vi "AlliGator Phasor Graph Panel.vi"() -> ()   [LabVIEW 2021, in "AlliGator Phasor Graph.lvlib"]
uses:
  AlliGator Phasor Graph.lvlib
  Phasor/Phasor Calibration Type.ctl
  Phasor/Phasor (g, s).ctl
  Phasor/Phasor (m, phi).ctl
  AlliGator Phasor Graph Ctrl Refnums.ctl
  Globals, Variables, Constants/AlliGator Refnums List.ctl
  Settings/AlliGator Settings List.ctl
  Action Engine/AlliGator Q Element.ctl
  Action Engine/AlliGator Q Event.ctl
  Graphs/XY Graph/XY Graph Event.ctl
  <vilib>/Utility/miscctls.llb/LVPoint32TypeDef.ctl
  Globals, Variables, Constants/AlliGator Variables List.ctl
  Variant/Variant to Data/Variant to Boolean.vi
  Settings/AlliGator Settings+.lvlib
  Variant/Variant to Data/Variant to Data.lvlib
  Notebook/Notebook.lvlib
  Action Engine/AlliGator Action Engine.lvlib
  GUI/GUI.lvlib
  GUI/AlliGator GUI.lvlib
  Error/Error.lvlib
  Graphs/XY Graph/XY Graph Add-Ons.lvlib
  Python Plugins API/AlliGator Python Plugins.lvlib
  Decay Analysis/Decay Processing/AlliGator Decay Processing.lvlib
  Phasor Calibration/AlliGator Phasor Calibration.lvlib
  Phasor/Phasor.lvlib
  Globals, Variables, Constants/AlliGator Globals, Variables & Constants.lvlib
  Utilities/Utilities.lvlib
panel:
  in  "Refresh SEPL":bool
  in  "Calibration Type":T1
  in  "Phasor Graph Active":bool
  in  "Phasor Graph Frequency":dbl[unit]=80000000.0 caption="Phasor Frequency"
  in  "Calibration Lifetime":dbl[unit] min=0.0
  in  "Pin Button":bool=TRUE
  out "Phasor Graph TipStrip":string caption="Lifetime Graph TipStrip"
  out "Phasor Graph":cluster{"X Array":dbl[], "Y Array":dbl[]}[](graph)
  in  "Phasor Reference 2 Control":dbl(c297)
  out "Phase Lifetime 2":dbl[unit]=nan format="%#.3g"
  out "Average Lifetime SDV":dbl[unit]=nan caption="+/-" format="%#.3g"
  out "Phasor Ratio SDV":dbl=nan caption="+/-" format="%#.3g"
  out "Modulus Lifetime SDV":dbl[unit]=nan caption="+/-" format="%#.3g"
  out "Phase Lifetime SDV":dbl[unit]=nan caption="+/-" format="%#.3g"
  out "Phasor Graph Average Lifetime":dbl[unit]=nan caption="<tau>_a" format="%#.3g"
  out "Phasor Graph Phasor Ratio":dbl=nan caption="Amplitude Ratio (a1)" format="%#.3g"
  out "Phasor Graph Modulus Lifetime":dbl[unit]=nan caption="Modulus Lifetime" format="%#.3g"
  in  "Current Phasor (m, phi)":T2={"m"=nan, "phi"=nan} {"phi" format="%#_4g"; "m" format="%#_4g"}
  in  "Phasor Reference 1 Control":dbl(c297)
  out "Phase Lifetime 1":dbl[unit]=nan format="%#.3g"
  out "Phasor Graph Phase Lifetime":dbl[unit]=nan caption="Phase Lifetime" format="%#.3g"
  in  "Current Phasor (g, s)":T3={"g"=nan, "s"=nan} caption="Current Phasor" {"s" format="%#_4g"; "g" format="%#_4g"}
  in  "Save Phasor Graph Image":bool
  in  "Single Step Phasor":bool
  in  "Phasor Frame Slide":i32(slide) caption="Phasor Frame Slider" min=0 step=1 scale=1.0..1.1
  in  "Show Line":bool
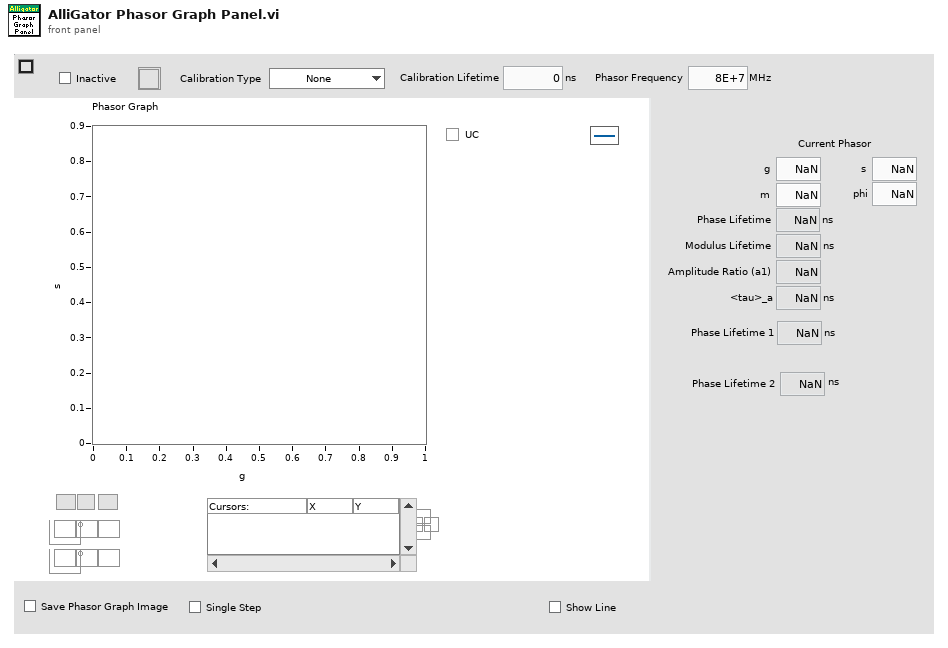
[diagram p1: front panel]
types:
  T1 = typedef "Phasor.lvlib/Phasor Calibration Type.ctl" = enum16{"None", "Single Phasor", "Phasor Series", "Phasor Map"}
  T2 = typedef "Phasor.lvlib/Phasor (m, phi).ctl" = cluster{"m":dbl, "phi":dbl}
  T3 = typedef "Phasor.lvlib/Phasor (g, s).ctl" = cluster{"g":dbl, "s":dbl}
  T4 = typedef "AlliGator GUI.lvlib/AlliGator Refnums List.ctl" = enum16{"---------- AlliGator Control Refnums ----------", "AlliGator Tab Control Refnum", "Dataset Ctrl Refnums", "Image Histogram Ctrl Refnums", "Intensity Time Trace Ctrl Refnums", "Decay Graph Ctrl Refnums", "Decay Statistics Graph Ctrl Refnums", "Phasor Graph Ctrl Refnums", "Phasor Ratio Graph Ctrl Refnums", "Phasor Plot Ctrl Refnums", "Lifetime & Other Parameters Ctrl Refnums", "Decay Fit Parameter Map Ctrl Refnums", "Parameter Map Ctrl Refnums", "Other AlliGator Ctrl Refnums", "---------- AlliGator Menu Refnums ----------", "AlliGator Menu", "---------- IO Device ID ----------", "Mouse ID", "Keyboard ID"}
  T5 = typedef "AlliGator Phasor Graph.lvlib/AlliGator Phasor Graph Ctrl Refnums.ctl" = cluster{"Phasor Ratio":refnum<vi>, "Modulus Lifetime":refnum<vi>, "Phasor at cursor (m, phi)":refnum<vi>, "Phase Lifetime":refnum<vi>, "Phasor at cursor (g, s)":refnum<vi>, "Phasor Graph Average Lifetime":refnum<vi>, "Phasor Graph Active":refnum<vi>, "Save Phasor Graph":refnum<vi>, "Phasor Frame Slide":refnum<vi>, "Single Step Phasor":refnum<vi>, "Calibration Type":refnum<vi>, "Show Line":refnum<vi>, "Phase Lifetime 1":refnum<vi>, "Phase Lifetime 2":refnum<vi>, "Phasor Graph Frequency":refnum<vi>, "Phasor Reference 1 Control":refnum<vi>, "Phasor Reference 2 Control":refnum<vi>, "Calibration Lifetime":refnum<vi>, "Phase Lifetime SDV":refnum<vi>, "Average Lifetime SDV":refnum<vi>, "Phasor Ratio SDV":refnum<vi>, "Modulus Lifetime SDV":refnum<vi>, "Phasor Graph":refnum<vi>}
  T6 = cluster{"Event Registration Refnum":refnum<event-registration>, "Event Registration Refnum":refnum<event-registration>}
  T7 = typedef "AlliGator Settings+.lvlib/AlliGator Settings List.ctl" = enum16{"GUI:Visible Settings Tab", "GUI:Last Run Version", "Source Image:Use Image Histogram for Contrast", "Source Image:Low Count Pixels Rejection Options", "Source Image:High Count Pixels Rejection Options", "Source Image:Use Image Brightness", "Source Image:Blend Overlay with Image Background", "Source Image:Use Fixed ROI Diameter", "Source Image:ROI Diameter", "Source Image:ROI Center Color", "Source Image:Peak Threshold", "Source Image:Intensity Threshold", "Source Image:Image Binning Options", "Source Image:Image Smoothing Options", "Source Image:Image Histogram Active", "Source Image:Invert Binary Mask", "Source Image:Hot Pixel Removal", "Source Image:Overlay Analyzed ROI Center", "Source Image:Auto-Adjust Contrast", "Source Image:Histogram Lower Percentile", "Source Image:Histogram Upper Percentile", "Source Image:Lock ROI with Maps", "Source Image:Save Source Image", "Source Image:Scale Bar Options", "Source Image:Image Resolution (Pixel Size)", "Source Image:Flatfield Correction", "Source Image:Show Dead Left Columns Correction", "Source Image:Dead Left Columns Correction", "Source Image:Image Pre-Processing Operations Order", "Source Image:Overlay ROI Median", "Source Image:Median Overlay Color", "Data Information:Gate Width", "Data Information:Nanotime Gate Separation", "Data Information:Macrotime Gate Separation", "Data Information:Gate Step", "Data Information:# Gates", "Data Information:Gate Image Exposure", "Data Information:Gate Image Integration", "Data Information:Gates to Skip", "Data Information:Gates to Keep", "Data Information:Define Gates to", "Data Information:Channel Name", "Data Information:Available Channel Names", "Data Information:Channel Arithmetic", "Data Information:Background File Subtraction", "Data Information:Background File", "Data Information:Background Scaling Factor", "Data Information:Background Pile-up Correction", "Data Information:Background Pixel Well Capacity", "Data Information:Laser Period", "Data Information:SYNC Period", "Data Information:Pile-up Correction", "Data Information:Pixel Well Capacity", "Data Information:Dataset Scaling Factor", "Fluorescence Decay_Decay Pre-Processing:Reverse Gates", "Fluorescence Decay_Decay Pre-Processing:Verbose Decay Pre-Processing", "Fluorescence Decay_Decay Pre-Processing:Use Decay Pre-Processing", "Fluorescence Decay_Decay Pre-Processing:Background Subtraction", "Fluorescence Decay_Decay Pre-Processing:Background Definition Range", "Fluorescence Decay_Decay Pre-Processing:Baseline Subtraction Method", "Fluorescence Decay_Decay Pre-Processing:Decay Pre-Processing Operations Order", "Fluorescence Decay_Decay Pre-Processing:Smoothing Parameter", "Fluorescence Decay_Decay Pre-Processing:Shift Decay", "Fluorescence Decay_Decay Pre-Processing:Decay Shift Parameters", "Fluorescence Decay_Decay Pre-Processing:Fold Decay", "Fluorescence Decay_Decay Pre-Processing:# Folds", "Fluorescence Decay_Decay Pre-Processing:1-Normalize Decay", "Fluorescence Decay_Decay Pre-Processing:[0-1]-Normalize Decay", "Fluorescence Decay_Decay Pre-Processing:Smoothen Decay", "Fluorescence Decay_Decay Pre-Processing:Extrapolate Decay", "Fluorescence Decay_Decay Pre-Processing:Use Periodicity", "Fluorescence Decay_Decay Pre-Processing:Use Cursors", "Fluorescence Decay_Decay Pre-Processing:Tail Fraction", "Fluorescence Decay_Decay Pre-Processing:Head Fraction", "Fluorescence Decay_Decay Pre-Processing:Additional Points", "Fluorescence Decay_Decay Pre-Processing:Straighten Decay", "Fluorescence Decay_Decay Pre-Processing:Constant Background", "Fluorescence Decay_Decay Pre-Processing:Pixel-Normalize Decay", "Fluorescence Decay_Advanced Analysis:Extract IRF instead of Decay", "Fluorescence Decay_Advanced Analysis:IRF Extraction Options", "Fluorescence Decay_Advanced Analysis:IRF Optimization Options", "Fluorescence Decay_Advanced Analysis:Square Pulse Options", "Fluorescence Decay_Advanced Analysis:IRF Order", "Fluorescence Decay_Advanced Analysis:IRF Time Constants", "Fluorescence Decay_Advanced Analysis:Wavelet Analysis Options", "Fluorescence Decay_Advanced Analysis:Average Lifetime Options", "Fluorescence Decay_Fit Options:Fit Options", "Fluorescence Decay_Fit Options:Use Legacy Fitting Approach", "Fluorescence Decay_Fit Options:Use Data Information Laser Period", "Fluorescence Decay_Fit Parameters:Displayed Fit Parameters", "Fluorescence Decay_Fit Parameters:Fit Parameter Constraints", "Fluorescence Decay_Fit Parameters:Export Tabulated Results", "Fluorescence Decay_Fit Parameters:MLE Baseline Offset Type", "Fluorescence Decay_Fit Parameters:MLE Baseline Offset", "Fluorescence Decay_Fit Parameters:Guess Parameter Names", "Fluorescence Decay_Fit Parameters:Guess Parameter Values", "Fluorescence Decay_Fit Parameters:Guess Parameters Options", "Fluorescence Decay_Fit Parameters:Optimal Offset Selection Criterion", "Fluorescence Decay_Styles:Show Last Decay Only", "Fluorescence Decay_Styles:Decay Graph Color Array", "Fluorescence Decay:Decay Graph Active", "Fluorescence Decay Statistics:Min Peak Value", "Fluorescence Decay Statistics:Reject Low Decay Peak Pixels", "Fluorescence Decay Statistics:Reject High Decay Peak Pixels", "Fluorescence Decay Statistics:Max Peak Value", "Time Traces:Use File Timestamp", "Time Traces:Time Step", "Time Traces:Use Intensity Correction File", "Time Traces:Intensity Correction File", "Phasor Plot:Phasor Plot Smoothing Options", "Phasor Plot:Phasor Plot Size", "Phasor Plot:Phasor Plot Graphics Options", "Phasor Plot:Cumulative Phasor Plot", "Phasor Plot:Use Phasor Brightness", "Phasor Plot:Blend Overlay with Phasor Background", "Phasor Plot:Save Phasor Plot", "Phasor Plot:Show References", "Phasor Plot:Phasor Ratio Decay Range", "Phasor Plot:Exponential Fading", "Phasor Plot:Phasor Ratio Reference Colors", "Phasor Plot:Reference Radius", "Phasor Plot:Show Color Map Vertices", "Phasor Plot:Phasor Plot Active", "Phasor Plot:Phasor Ratio Color Map Type", "Phasor Plot:Phasor Ratio Color Map", "Phasor Plot:Phasor Ratio Display Range", "Phasor Plot:Selected Image ROI(s)", "Phasor Plot:All Image ROIs", "Phasor Plot:Selected Phasor Plot ROI(s)", "Phasor Plot:All Phasor Plot ROIs", "Phasor Plot:Phasor Ratio Color-Coded Quantity", "Phasor Plot:Store Phasor Harmonics", "Phasor Plot:Draw Reference Segment", "Phasor Plot:User-Defined Quantity", "Phasor Plot:Color Scale High Color", "Phasor Plot:Color Scale Low Color", "Phasor Plot:Intensity-weighted Phasor Plot", "Phasor Graph:Phasor Frequency", "Phasor Graph:Phasor Ratio Type", "Phasor Graph:Pixel-level Phasor Computation", "Phasor Graph:Save Phasor Graph", "Phasor Graph:Phasor Graph Active", "Phasor Graph:Phasor SDV Options", "Phasor Graph:Intensity-weighted Phasor Graph", "Phasor Graph:Define Shortest Lifetime as", "Phasor Calibration:Use Backup Calibration if needed", "Phasor Calibration:Backup Calibration Type", "Phasor Calibration:Calibration Type", "Phasor Calibration:Calibration Lifetime", "Phasor Calibration:Calibration Map Algorithm", "Single-Exponential Phasor Locus (SEPL):Gate Parameters", "Single-Exponential Phasor Locus (SEPL):User-defined Gate", "Single-Exponential Phasor Locus (SEPL):User-defined IRF", "Single-Exponential Phasor Locus (SEPL):Phasor Parameters", "Single-Exponential Phasor Locus (SEPL):Decay & IRF Parameters", "Single-Exponential Phasor Locus (SEPL):Display Parameters", "Lifetime Analysis:Decay Analysis Parameters", "Lifetime Analysis:Lifetime Map Active", "Plugins:Python Settings", "Miscellaneous:Verbose Mode", "Miscellaneous:Beep after Script", "Miscellaneous:Saved Image File Format", "Miscellaneous:Exported Gate Image Settings", "Miscellaneous:Include Loading in Timing", "Miscellaneous:Verbose Settings Mode", "Miscellaneous:Histogram Options", "Miscellaneous:Beep on Error", "Miscellaneous:# Logical Processors Used", "Miscellaneous:ROI Description Max Characters", "Miscellaneous:Verbose Error Mode", "Miscellaneous:Transparent Mask Color"}
  T8 = typedef "AlliGator Action Engine.lvlib/AlliGator Q Element.ctl" = cluster{"AlliGator Q Event":T9, "Data":variant}
  T9 = typedef "AlliGator Action Engine.lvlib/AlliGator Q Event.ctl" = enum16{"---- Files ----", "Files:Set Batch Export Files To Save", "Files:Set Dataset Loading & Pre-processing Options", "Files:Check #Frames in Dataset", "Files:Increment Frame Index", "Files:Open Mask Image", "Files:Open White Light Image", "Files:Open Single Dataset", "Files:New Folder of Folders Selected", "Files:Load File (all Types)_Scriptable", "Files:Move Flattened Series to Folders Series", "Files:Select Folder", "Files:Load FLI Dataset", "Files:Load Swiss SPAD 1 Dataset", "Files:Load Swiss SPAD 2 Dataset", "Files:Load .sdt FLI Dataset", "Files:Load .ptu FLI Dataset", "Files:Load .bin FLI Dataset", "Files:Load Single Gate Image Folder", "Files:Load I/m/phi Dataset (deprecated)", "Files:Load Single Image", "Files:Subtract Background File", "Files:Export FLI Dataset", "Files:Load HDF5 FLI Dataset", "Files:Set Destination File Path", "Files:Save Mask Image", "Files:Batch Conversion", "Files:New Folder Selected", "Files:Close FLI Dataset", "Files:Close FLI Dataset Series", "Files:Close White Light Image", "Files:Close Mask Image", "---- FLI Dataset ----", "FLI Dataset:Channel Arithmetic", "FLI Dataset:Export Average Lifetime Map as ASCII", "FLI Dataset:Export User-Defined Quantity Map as ASCII", "FLI Dataset:Python Function FLI Dataset Event", "FLI Dataset:ROI Analysis", "FLI Dataset:Tilted Logistic Square Gated IRF Characteristics Map", "FLI Dataset:Logistic Square Gated IRF Characteristics Map", "FLI Dataset:Square Gated IRF Characteristics Map", "FLI Dataset:Multi-ROI Single-Pixel Phasor Analysis", "FLI Dataset:Multi-ROI Single-Pixel NLSF Analysis", "FLI Dataset:All ROIs IRF Extraction", "FLI Dataset:All ROIs Decay Fit Non-Interactive (Fast + Individual IRF)", "FLI Dataset:All ROIs Phasor Analysis", "FLI Dataset:All ROIs Decay Fit", "FLI Dataset:Fluorescence Decay Statistics", "FLI Dataset:Update Decay Statistics Graph", "FLI Dataset:Get Decay from ROI", "FLI Dataset:All ROIs Average Lifetimes", "FLI Dataset:Save/Load Local IRFs", "FLI Dataset:Clear Local IRFs", "FLI Dataset:Phasor Calibration Maps (# Gates Series) Script", "FLI Dataset:Calibrated Phasor Map Series", "---- FLI Dataset Series ----", "FLI Dataset Series:Sum All Datasets in Series", "FLI Dataset Series:Add Dataset to Accumulated Dataset", "FLI Dataset Series:Display Accumulated Dataset", "FLI Dataset Series:Clear Dataset Series Sum", "FLI Dataset Series:Time-Series Analysis (NLSF)", "FLI Dataset Series:Time-Series Analysis (Phasor)", "---- Image ----", "Image:Update Image Profile Plots", "Image:Image Histogram Cursor Move", "Image:Image Histogram", "Image:Image Contrast", "Image:Set Image Histogram Cursor Move Flag", "Image:Clear Image Overlay", "Image:Use ROI as Search Area", "Image:Set ROI Diameter", "Image:Save Image Data as TIFF", "Image:Save Displayed Image with Overlay", "Image:Save Image Overlay Only", "Image:Save Image as Hot Pixel Mask", "Image:Change Source Image Color Palette", "Image:Copy Image to Clipboard", "Image:Source Image ROI Selection", "Image:Delete All ROIs", "Image:Delete All Unselected ROIs", "Image:Delete ROI", "Image:Merge All ROIs", "Image:Store ROI", "Image:Source Image ROI Storage", "Image:Export ROI Description to Notebook", "Image:Save ROI", "Image:Load ROI", "Image:Paste ROI Definition", "Image:Clear ROI", "Image:Identify ROIs in Mask Image", "Image:Create Complementary ROI", "Image:Create Contour ROI", "Image:Create ROI(s) from Pixels with Peak above Min_Scriptable", "Image:Create ROI(s) from Pixels with Intensity above Min_Scriptable", "Image:Compute ROI Statistics", "Image:Delete ROI(s) based on ROI Characteristics", "Image:Create ROI Grid", "Image:ROI to Individual Pixel ROIs", "Image:Python Function Source Image Event", "Image:Show Phasor Calibration Map ROI Centers", "Image:Convert ROI to Mask Image", "Image:Mouse Move", "Image:Mouse Up", "Image:Set Source Image Mouse Move Flag", "Image:Add Scale Bar Overlay", "Image:Delete Existing ROIs Option", "Image:Overlay ROI Median", "Image:Check Current ROI", "Image:Update True Pixel Value", "Image:Use ROI", "---- Decay ----", "Decay:Clear IRF/Reference Plot", "Decay:Add Decay to Graph", "Decay:Smoothen Plot", "Decay:Smoothen Plot Tail", "Decay:Average Selected Plots", "Decay:Extract IRF", "Decay:Optimal IRF Extraction", "Decay:Threshold IRF", "Decay:Fit to Model IRF", "Decay:Fit IRF to Square Gate", "Decay:Fit IRF to Logistic Square Gate", "Decay:Fit IRF to Tilted Logistic Square Gate", "Decay:Create Bounding Cursors Set", "Decay:Export Bounding Cursors Definition to Notebook", "Decay:Denoise Plot", "Decay:Compute Cumulative Function", "Decay:Use as Reference Decay", "Decay:Show Reference Decay/IRF", "Decay:Extrapolate Decay", "Decay:Create Head & Tail Bounding Cursors", "Decay:Store Cursor-defined Head & Tail Fractions", "Decay:Rebin Plot", "Decay:1-Normalize Decay", "Decay:[0-1]-Normalize Plot", "Decay:Straighten Decay", "Decay:Shift Decay", "Decay:Fold Decay", "Decay:Fit Decay", "Decay:Global Fit of Selected Decays", "Decay:Post Global Fit Script", "Decay:Add Global Fit Parameters to Graph", "Decay:Add Decay Parameter(s) to Plot (Graph)", "Decay:Export Decay to Phasor Graph", "Decay:Compute Average Lifetime", "Decay:Plot Convolution", "Decay:Graph Tip Strip Update", "---- Decay Statistics ----", "Decay Statistics:Tip Strip Update", "---- Intensity Time Trace ----", "Intensity Time Trace:Use File Timestamp", "Intensity Time Trace:Load Intensity Corrections File", "Intensity Time Trace:Clear Intensity Corrections File", "Intensity Time Trace:Tip Strip Update", "---- Phasor Plot ----", "Phasor Plot:Build Phasor Plot", "Phasor Plot:Change Phasor Plot Color Palette", "Phasor Plot:Adjust Phasor Plot Display Range", "Phasor Plot:Highlight Image ROI in Phasor Plot", "Phasor Plot:Save Phasor Plot Image with Overlay", "Phasor Plot:Export Complex Phasor Map", "Phasor Plot:Export Phasor Ratio Map", "Phasor Plot:Export Average Lifetime Map", "Phasor Plot:Compute Phase Lifetime Histogram", "Phasor Plot:Compute Phasor Ratio Histogram", "Phasor Plot:Compute Phase Lifetime vs Intensity Scatter Plot", "Phasor Plot:Weber 2-Component Decomposition", "Phasor Plot:Update Phasor Color Map Vertices", "Phasor Plot:Clear Phasor Overlay", "Phasor Plot:Use Segment Extremities as References", "Phasor Plot:Use UC/Segment Intersections as References", "Phasor Plot:Use UC/Principal Axis Intersections as References", "Phasor Plot:Use UC/Linear Fit Intersections as References", "Phasor Plot:Update Phasor Plot Reference", "Phasor Plot:Show Local Phasor Info in Phasor Plot", "Phasor Plot:Update Phasor Plot State", "Phasor Plot:Phasor Plot ROI Storage", "Phasor Plot:Phasor Plot ROI Selection", "Phasor Plot:Python Function Phasor Plot Event", "Phasor Plot:Overlay Phasor ROI, Ratio or Map in Source Image", "Phasor Plot:Compute Decay of Selected Phasors", "Phasor Plot:Phasor at Image Pixel", "Phasor Plot:Mouse Move", "Phasor Plot:Mouse Up", "Phasor Plot:Display Range Mouse Move", "Phasor Plot:Set Mouse Move Flag", "Phasor Plot:Update True Phasor Plot Value", "---- Phasor Graph ----", "Phasor Graph:Get Phasor Value", "Phasor Graph:Create New Phasor Plot Dialog", "Phasor Graph:Update Last Phasor Value", "Phasor Graph:Update Phasor (m, phi)", "Phasor Graph:Remove Single Phasor from Plot", "Phasor Graph:Add Single Phasor to Plot", "Phasor Graph:Remove Phasor Plot", "Phasor Graph:Remove Selected Phasor Plots", "Phasor Graph:Clear Phasor Data", "Phasor Graph:Clear Phasor Graph", "Phasor Graph:Cursor Move", "Phasor Graph:Draw Cursor Connecting Line", "Phasor Graph:Clear Cursor Connecting Line", "Phasor Graph:Find UC Intersection", "Phasor Graph:Use UC/Cursor-Defined Line Intersections", "Phasor Graph:Use Selected Plots Fitted Line/UC Intersections", "Phasor Graph:Use Selected Plots Principal Axis/UC Intersections", "Phasor Graph:Show Single Phasor", "Phasor Graph:Save Single Phasor Plot", "Phasor Graph:Save All Phasor Plots", "Phasor Graph:Load Phasor Plot(s)", "Phasor Graph:Phasor Multiplication", "Phasor Graph:Compute Average Phasor", "Phasor Graph:Compute Multiple Average Phasors (Selected Plots)", "Phasor Graph:Export Single Phasor Plot Phase Lifetimes", "Phasor Graph:Parameter 2 vs Parameter 1 Scatter Plot", "Phasor Graph:Use Cursor n Location", "Phasor Graph:Set Reference n to Current Phase Lifetime Value", "Phasor Graph:Set Reference n to Lifetime Value", "Phasor Graph:Set Cursor n Location", "Phasor Graph:Save Phasor Graph Image", "Phasor Graph:Update SEPL Plot", "Phasor Graph:Export Single Phasor Plot Data", "Phasor Graph:Export Selected Phasor Plots Data", "Phasor Graph:Python Function Phasor Graph Event", "Phasor Graph:Tip Strip Update", "---- Calibration ----", "Calibration:Set Calibration Type", "Calibration:Load/Save Phasor Calibration", "Calibration:Load/Save Phasor Calibration Series", "Calibration:Load/Save Phasor Calibration Map", "Calibration:Use as Calibration", "Calibration:Compute Optimal Calibration from Phasor References", "Calibration:Clear Phasor Calibration", "Calibration:Single Phasor Calibration Information", "Calibration:Use as Calibration Series", "Calibration:Use as Calibration Map", "Calibration:Clear Calibration Series", "Calibration:Phasor Calibration Series Information", "Calibration:Clear Calibration Map", "Calibration:Phasor Calibration Map Information", "Calibration:Apply Phasor Calibration", "Calibration:Update Single Plot Calibration", "Calibration:Update Multiple Plots Calibration", "Calibration:Clear Single Plot Calibration", "Calibration:Clear All Plots Calibrations", "Calibration:Clear Plot(s) Calibration(s)?", "---- Phasor Ratio ----", "Phasor Ratio:Clear Reference n", "Phasor Ratio:Toggle Selected Plot(s)  Lock to Reference 1", "Phasor Ratio:Use as Reference n", "Phasor Ratio:Send Reference n to Notebook", "Phasor Ratio:Toggle Selected Plot(s)  Lock to Reference 2", "Phasor Ratio:Compute Phasor Ratio at Mouse Location", "Phasor Ratio:Compute Phasor Plot's Average Phasor Ratio", "Phasor Ratio:Compute Time-Series Phasor Ratios", "Phasor Ratio:Fit Line to Phasor Ratio Plot", "Phasor Ratio:Save References", "Phasor Ratio:Load References", "Phasor Ratio:Update Phasor Reference 1", "Phasor Ratio:Update Phasor Reference 2", "Phasor Ratio:Move Cursor n to Reference n", "Phasor Ratio:Use as Phasor Reference 1 Lifetime", "Phasor Ratio:Use as Phasor Reference 2 Lifetime", "Phasor Ratio:Export Phasor Ratio Map as ASCII", "Phasor Ratio:Tip Strip Update", "---- Lifetime & Other Parameters Graph ----", "Lifetime:Compute Sliced Mean, SDV and CV Plots", "Lifetime:Plot Decay Shifts", "Lifetime:Plot Histogram", "---- Decay Fit Parameter Map ----", "Decay Fit Parameter Map:Export ROI NLSF Data as ASCII", "Decay Fit Parameter Map:Set Decay Fit Parameter Map Selection", "Decay Fit Parameter Map:Build Decay Fit Parameter Map", "Decay Fit Parameter Map:Change Decay Fit Parameter Map Color Palette", "Decay Fit Parameter Map:Export Decay Fit Parameter Map Data as ASCII", "Decay Fit Parameter Map:Export All Decay Fit Parameter Maps Data as ASCII", "Decay Fit Parameter Map:Selected Parameter Scatterplot", "Decay Fit Parameter Map:Parameter 2 vs Parameter 1 Scatterplot", "Decay Fit Parameter Map:Save Decay Fit Parameter Map Image", "Decay Fit Parameter Map:Save-Load IRFs & Fit Data", "Decay Fit Parameter Map:Update Local Decay Plots", "Decay Fit Parameter Map:Python Function Decay Fit Parameters Map Event", "Decay Fit Parameter Map:Overlay Decay Fit Parameter Map in Source Image", "Decay Fit Parameter Map:Selected Parameter vs Intensity Scatterplot", "Decay Fit Parameter Map:Mouse Up", "Decay Fit Parameter Map:Mouse Move", "Decay Fit Parameter Map:Display Range Mouse Move", "Decay Fit Parameter Map:Change Map Resolution", "Decay Fit Parameter Map:Variance Significance Maps", "Decay Fit Parameter Map:Fit Result Constraints Window", "Decay Fit Parameter Map:Use ROI", "---- Parameter Map ----", "Parameter Map:Export ROI Parameters Data as ASCII", "Parameter Map:Add Parameter Map Set", "Parameter Map:Delete Parameter Map Set", "Parameter Map:Update Parameter List", "Parameter Map:Build Parameter Map", "Parameter Map:Change Parameter Map Color Palette", "Parameter Map:Export Parameter Map Data as ASCII", "Parameter Map:Export All Parameter Maps Data as ASCII", "Parameter Map:Selected Parameter Scatterplot", "Parameter Map:Parameter 2 vs Parameter 1 Scatterplot", "Parameter Map:Selected Parameter vs Intensity Scatterplot", "Parameter Map:Save Parameter Map Image", "Parameter Map:Save-Load IRFs & Parameter Maps (TODO)", "Parameter Map:Set Parameter Map Selection", "Parameter Map:Python Function Parameter Map Event", "Parameter Map:Overlay Parameter Map in Source Image", "Parameter Map:Update Local Decay Plots", "Parameter Map:Mouse Up", "Parameter Map:Mouse Move", "Parameter Map:Display Range Mouse Move", "Parameter Map:Use ROI", "---- Generic Graph ----", "Generic Graph:Generic XY Graph Event", "Generic Graph:Python Function XY Graph Event", "Generic Graph:New Plot", "Generic Graph:Save Plot", "Generic Graph:XY Plot Histogram", "Generic Graph:Set XY Graph Plot Name", "Generic Graph:Set Last Cursor Style", "Generic Graph:Tip Strip Update", "---- GUI ----", "GUI:Start Script", "GUI:Type of Displayed Image Changed", "GUI:Gate Image Slide Changed", "GUI:Show Busy Icon", "GUI:Show Busy Icon & Abort Button", "GUI:Hide Busy Icon", "GUI:Hide Busy Icon & Abort Button", "GUI:Abort", "GUI:End Script", "GUI:Start Timing", "GUI:End Timing", "GUI:Set State Indicator", "GUI:Send Parameters JSON Strings to Clipboard", "GUI:Set Gate Step", "GUI:Idle", "GUI:Initialization", "GUI:Quit", "GUI:Increment Dataset Index", "GUI:Set Dataset Index to -1", "GUI:Time Series Slider Moved", "GUI:Time Series Slider Changed", "GUI:Toggle Playback or Loop", "GUI:Playback Script", "GUI:Set Phasor Frequency", "GUI:Open Window", "GUI:Start Test Script", "GUI:End Test Script", "GUI:Set Verbose Mode", "GUI:Set Verbose Settings Mode", "GUI:Initialize Python Session", "DEBUG"}
  T10 = typedef "AlliGator Globals, Variables & Constants.lvlib/AlliGator Variables List.ctl" = enum16{"---- GUI ----", "GUI:Initialization Status", "GUI:State Indicators Refnum", "GUI:Original AlliGator Menu Items", "GUI:Current Action Loop State", "GUI:Script in progress", "GUI:Playback", "GUI:Loop Playback", "GUI:Search ROI Used", "GUI:Search ROI", "Image Histogram Max Legend Size", "Decay Graph Max Legend Size", "Intensity Graph Max Legend Size", "Decay Statistics Graph Max Legend Size", "Phasor Graph Max Legend Size", "Phasor Ratio Graph Max Legend Size", "Lifetime Graph Max Legend Size", "---- Files ----", "Files:Export Dataset Frames as Individual Files", "Files:Show Batch Export Help Balloons", "Files:Frames in Dataset", "Files:ptu File Frame Start Indices", "Files:Current Frame in Dataset", "Files:Current Frame Timestamp", "Files:Dataset Loaded", "Files:Dataset Metadata", "Files:Dataset Channel", "Files:Dataset Data Description", "Files:Background Dataset Metadata", "Files:Background Dataset Channel", "Files:Background Dataset Data Description", "Files:Background File Subtraction", "Files:Background File Path", "Files:Background File Pile-up Correction", "Files:Background File Pixel Well Capacity", "Files:Background File Scaling Factor", "Files:Current Dataset Load Settings", "Files:Dataset Path", "Files:ICCD-specific Information", "Files:Macrotime Gate Separation", "------ Python Plugins ------", "Python Plugins:Information", "Python Plugins:Python Session", "Python Plugins:Valid Python Session?", "---- Source Image ----", "Source Image:ROIs", "Source Image:Current ROI", "Source Image:ROI Event Refnum", "X_Source Image:Display Range", "X_Source Image:Palette Information", "X_Source Image:Type of Displayed Image", "X_Time Gate Slider", "Source Image:Palette List", "Source Image:Scale", "Source Image:ROI Overlay Color", "Source Image:Overlay to Erase", "Source Image:Is Displayed Image Accumulated", "Source Image:White Light Image Modified", "Source Image:Mask Image Modified", "---- Image Profile Window ----", "Image Profile:Window Event Refnum", "Image Profile:IntensityType", "Image Profile:Intensity Average Type", "Image Profile:Intensity-weighted SDV", "Image Profile:Box Profile Type", "Image Profile:Window Open", "Image Profile:Plotted Fit Parameter", "------ Phasor Graph -------", "Phasor Graph:Show Line", "---- Phasor Plot ---", "Phasor Plot:Parameters Changed", "Phasor Plot:FLI Dataset Modified since last Calculation", "Phasor Harmonics Data", "Selected Phasor Harmonics", "Phasor Harmonic Manager Event Refnum", "Phasor Plot:ROIs", "Phasor Plot:Current ROI", "Phasor Plot:ROI Event Refnum", "Phasor Plot:Image Reference Points", "Phasor Plot:Computed", "Phasor Plot:Palette Information", "Phasor Plot:Palette List", "Phasor Plot:Phasor Ratio Palette Information", "Phasor Plot:Phasor Ratio Palette List", "Phasor Plot:Image Scale", "Phasor Plot:Image Overlay to Erase", "Phasor Plot:Image Elements to Update", "Phasor Plot:Current Calculation Parameters", "Phasor Plot:Current Calibration Options", "Phasor Plot:Reset Cumulated Phasor Plot", "Phasor Plot:Reference 1", "Phasor Plot:Lifetime Reference 1", "Phasor Plot:Reference 1 Frequency", "Phasor Plot:Reference 2", "Phasor Plot:Lifetime Reference 2", "Phasor Plot:Reference 2 Frequency", "---- Decay Analysis ----", "Number of Selected Decays to Fit", "LS Fit Results", "LAR Fit Results", "BS Fit Results", "Last Decay Max - Min", "Best Fit Parameters", "Best Fit Parameter Names", "Actual Size X", "Actual Size Y", "Binning X", "Binning Y", "Actual # Gates", "Dataset Number", "Gates to...", "Gates Skipped", "Gates to keep", "Gate Step", "Gate Separation", "Reversed Gates", "Pile-up Correction", "Pixel Well Capacity", "Background Subtracted", "Background Subtraction Method", "Background Definition Range", "Background File (deprecated)", "Number of Dataset Accumulated", "Array of Accumulated Dataset Paths", "Do Averaged Datasets", "Destination File Path", "Process Plot Target", "Use 1/D as Phasor Frequency", "---- Decay Fit Parameter Map -----", "Decay Fit Parameter Map:Palette Information", "Decay Fit Parameter Map:Palette List", "Decay Fit Parameter Map:X Resolution", "Decay Fit Parameter Map:Y Resolution", "Decay Fit Parameter Map:Use Decay Fit Result Constraints", "Decay Fit Parameter Map:Decay Fit Result Constraints", "Decay Fit Parameter Map:Decay Fit Result Constraints Applied", "---- Parameter Map ----", "Parameter Map:Palette Information", "Parameter Map:Palette List", "------- Local Decay Window ---------", "Local Decay Graph Window:Event Refnum", "Local Decay Graph Window:Use normalized IRF for convolution", "----- Miscellaneous ----", "Misc:Skippable Dialog Windows Status"}
  T11 = typedef "XY Graph Add-Ons.lvlib/XY Graph Event.ctl" = cluster{"Item Tag":string, "XY Graph Refnum":refnum<vi>, "Coords":T12, "Item Path":string}
  T12 = typedef "LVPoint32TypeDef.ctl" = cluster{"Horizontal":i32, "Vertical":i32}
  T13 = enum16{"0", "1", "2", "3", "4", "5", "6", "7", "8", "9", "A", "B", "C", "D", "E", "F", "G", "H", "I", "J", "K", "L", "M", "N", "O", "P", "Q", "R", "S", "T", "U", "V", "W", "X", "Y", "Z", "F1", "F2", "F3", "F4", "F5", "F6", "F7", "F8", "F9", "F10", "F11", "F12", "F13", "F14", "F15", "ADD", "BACK", "BACKSLASH", "CAPITAL", "COMMA", "DECIMAL", "DELETE", "DIVIDE", "DOWN", "END", "EQUALS", "ESCAPE", "GRAVE (`)", "HOME", "INSERT", "LBRACKET", "LCONTROL", "LEFT", "L ALT", "LSHIFT", "LWIN", "MINUS", "MULTIPLY", "NEXT", "NUMLOCK", "NUMPAD_0", "NUMPAD_1", "NUMPAD_2", "NUMPAD_3", "NUMPAD_4", "NUMPAD_5", "NUMPAD_6", "NUMPAD_7", "NUMPAD_8", "NUMPAD_9", "PAUSE", "PERIOD", "PRIOR (PG UP)", "RBRACKET", "RCONTROL", "RETURN", "RIGHT", "R ALT", "RSHIFT", "RWIN", "SCROLL", "SEMICOLON", "SLASH", "SPACE", "SUBTRACT", "TAB", "UP", "ENTER (num pad)", "' (quote)"}
  T14 = typedef "XY Graph Add-Ons.lvlib/XY Graph Refnum.ctl" = refnum<vi>
  T15 = enum16{"0", "1", "2", "3", "4", "5", "6", "7", "8", "9", "A", "B", "C", "D", "E", "F", "G", "H", "I", "J", "K", "L", "M", "N", "O", "P", "Q", "R", "S", "T", "U", "V", "W", "X", "Y", "Z", "F1", "F2", "F3", "F4", "F5", "F6", "F7", "F8", "F9", "F10", "F11", "F12", "F13", "F14", "F15", "ADD", "BACK", "BACKSLASH", "CAPITAL", "COMMA", "DECIMAL", "DELETE", "DIVIDE", "DOWN", "END", "EQUALS", "ESCAPE", "GRAVE (`)", "HOME", "INSERT", "LBRACKET", "LCONTROL", "LEFT", "L ALT", "LSHIFT", "LWIN", "MINUS", "MULTIPLY", "NEXT", "NUMLOCK", "NUMPAD_0", "NUMPAD_1", "NUMPAD_2", "NUMPAD_3", "NUMPAD_4", "NUMPAD_5", "NUMPAD_6", "NUMPAD_7", "NUMPAD_8", "NUMPAD_9", "PAUSE", "PERIOD", "PRIOR (PG UP)", "RBRACKET", "RCONTROL", "RETURN", "RIGHT", "R ALT", "RSHIFT", "RWIN", "SCROLL", "SEMICOLON", "SLASH", "SPACE", "SUBTRACT", "TAB", "UP", "ENTER (num pad)", "' (quote)"}[]
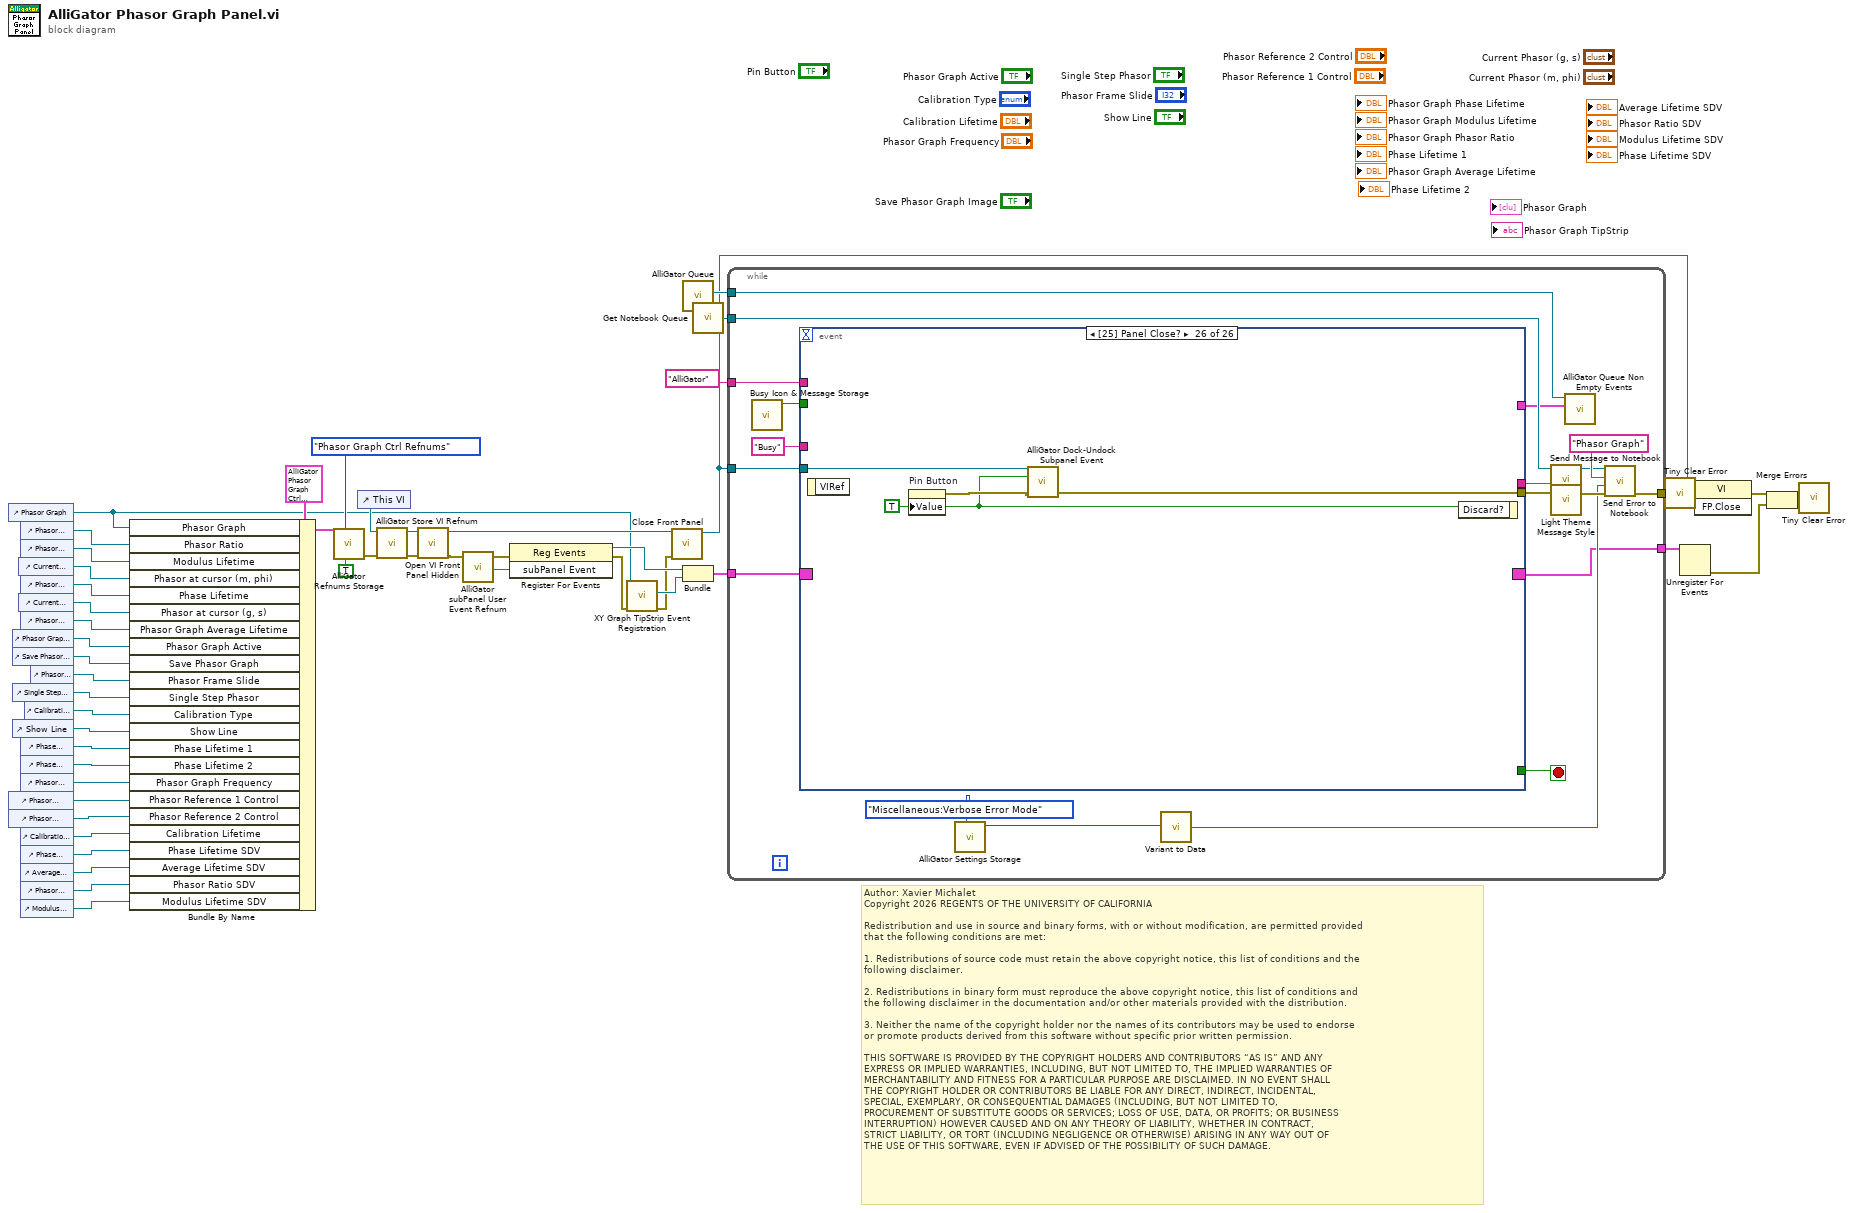
[diagram p0: block diagram]
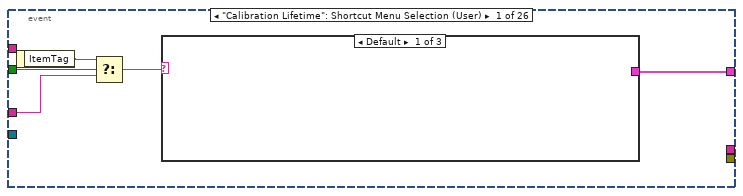
[diagram p2: hidden frame]
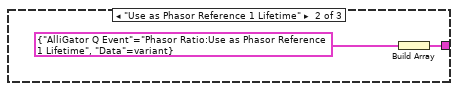
[diagram p3: hidden frame]
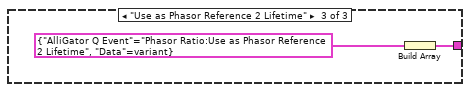
[diagram p4: hidden frame]
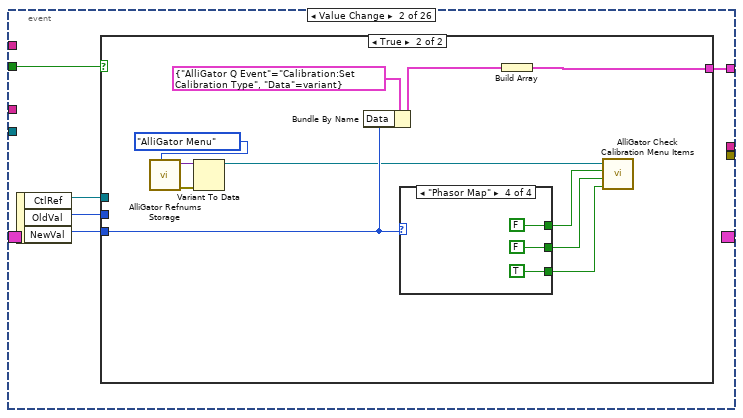
[diagram p5: hidden frame]
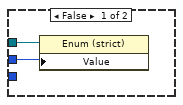
[diagram p6: hidden frame]
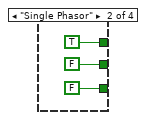
[diagram p8: hidden frame]
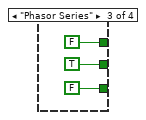
[diagram p9: hidden frame]
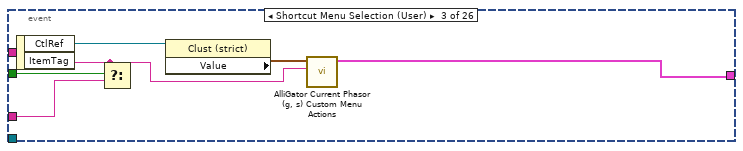
[diagram p10: hidden frame]
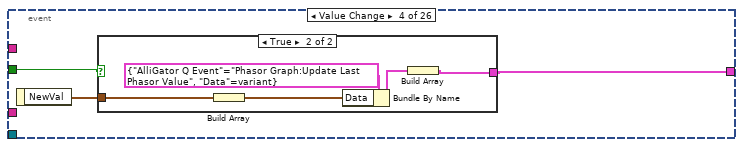
[diagram p11: hidden frame]
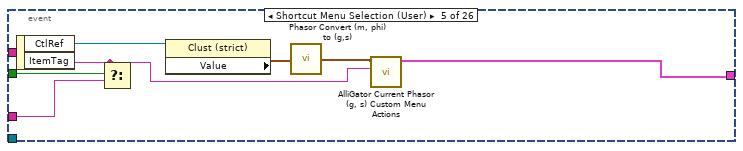
[diagram p13: hidden frame]
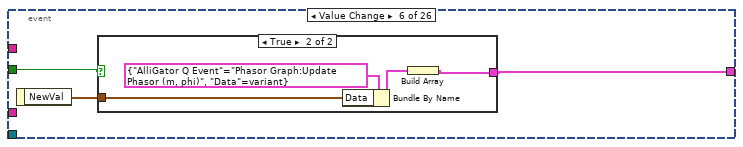
[diagram p14: hidden frame]
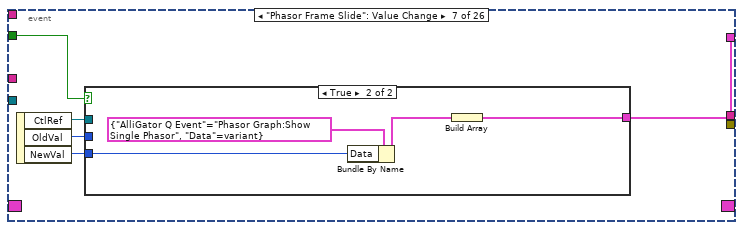
[diagram p16: hidden frame]
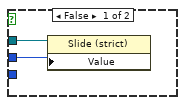
[diagram p17: hidden frame]
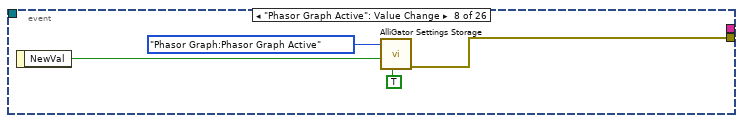
[diagram p18: hidden frame]
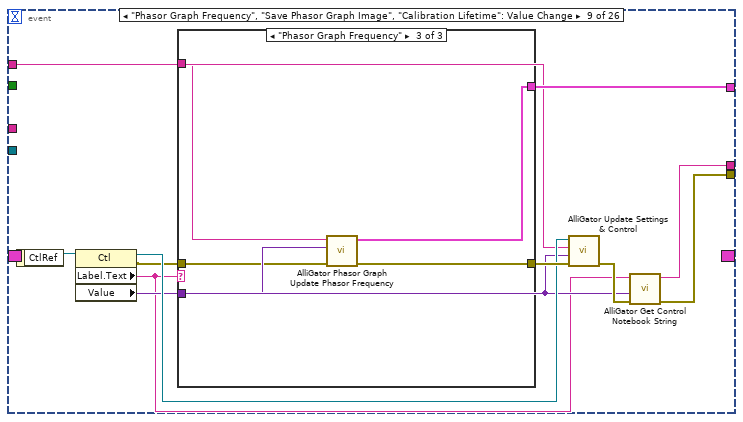
[diagram p19: hidden frame]
diagram:
  # "Author: Xavier Michalet\nCopyright 2026 REGENTS OF THE UNIVERSITY OF CALIFORNIA\n\nRedistribution and use in source and binary forms, with or without modification, are permitted provided\nthat the following conditions are met:\n\n1. Redistributions of source code must retain the above copyright notice, this list of conditions and the\nfollowing disclaimer.\n\n2. Redistributions in binary form must reproduce the above copyright notice, this list of conditions and\nthe following disclaimer in the documentation and/or other materials provided with the distribution.\n\n3. Neither the name of the copyright holder nor the names of its contributors may be used to endorse \nor promote products derived from this software without specific prior written permission.\n\nTHIS SOFTWARE IS PROVIDED BY THE COPYRIGHT HOLDERS AND CONTRIBUTORS “AS IS” AND ANY \nEXPRESS OR IMPLIED WARRANTIES, INCLUDING, BUT NOT LIMITED TO, THE IMPLIED WARRANTIES OF\nMERCHANTABILITY AND FITNESS FOR A PARTICULAR PURPOSE ARE DISCLAIMED. IN NO EVENT SHALL\nTHE COPYRIGHT HOLDER OR CONTRIBUTORS BE LIABLE FOR ANY DIRECT, INDIRECT, INCIDENTAL, \nSPECIAL, EXEMPLARY, OR CONSEQUENTIAL DAMAGES (INCLUDING, BUT NOT LIMITED TO, \nPROCUREMENT OF SUBSTITUTE GOODS OR SERVICES; LOSS OF USE, DATA, OR PROFITS; OR BUSINESS\nINTERRUPTION) HOWEVER CAUSED AND ON ANY THEORY OF LIABILITY, WHETHER IN CONTRACT, \nSTRICT LIABILITY, OR TORT (INCLUDING NEGLIGENCE OR OTHERWISE) ARISING IN ANY WAY OUT OF\nTHE USE OF THIS SOFTWARE, EVEN IF ADVISED OF THE POSSIBILITY OF SUCH DAMAGE."
  n1 = control-ref of="Phasor Graph"() -> (w1:refnum<vi>)
  n2 = control-ref of="Phasor Reference 1 Control"() -> (w11:refnum<vi>)
  n3 = control-ref of="Phasor Reference 2 Control"() -> (w17:refnum<vi>)
  n4 = control-ref of="Phasor Graph Active"() -> (w26:refnum<vi>)
  n5 = control-ref of="Save Phasor Graph Image"() -> (w25:refnum<vi>)
  n6 = control-ref of="Single Step Phasor"() -> (w23:refnum<vi>)
  n7 = control-ref of="Show Line"() -> (w21:refnum<vi>)
  n8 = control-ref of="Current Phasor (m, phi)"() -> (w30:refnum<vi>)
  n9 = control-ref of="Current Phasor (g, s)"() -> (w28:refnum<vi>)
  n10 = control-ref of="Phasor Graph Phasor Ratio"() -> (w32:refnum<vi>)
  n11 = control-ref of="Phasor Graph Modulus Lifetime"() -> (w31:refnum<vi>)
  n12 = control-ref of="Phasor Graph Phase Lifetime"() -> (w29:refnum<vi>)
  n13 = control-ref of="Phasor Graph Average Lifetime"() -> (w27:refnum<vi>)
  n14 = control-ref of="Phase Lifetime 1"() -> (w20:refnum<vi>)
  n15 = control-ref of="Phase Lifetime 2"() -> (w19:refnum<vi>)
  n16 = control-ref of="Phasor Graph Frequency"() -> (w18:refnum<vi>)
  n17 = control-ref of="Calibration Lifetime"() -> (w16:refnum<vi>)
  n18 = control-ref of="Phase Lifetime SDV"() -> (w15:refnum<vi>)
  n19 = control-ref of="Average Lifetime SDV"() -> (w14:refnum<vi>)
  n20 = control-ref of="Phasor Ratio SDV"() -> (w13:refnum<vi>)
  n21 = control-ref of="Modulus Lifetime SDV"() -> (w12:refnum<vi>)
  n22 = control-ref of="Calibration Type"() -> (w22:refnum<vi>)
  n23 = control-ref of="Phasor Frame Slide"() -> (w24:refnum<vi>)
  n24 = Bundle By Name(cluster=T5 {"Phasor Ratio"=refnum, "Modulus Lifetime"=refnum, "Phasor at cursor (m, phi)"=refnum, "Phase Lifetime"=refnum, "Phasor at cursor (g, s)"=refnum, "Phasor Graph Average Lifetime"=refnum, "Phasor Graph Active"=refnum, "Save Phasor Graph"=refnum, "Phasor Frame Slide"=refnum, "Single Step Phasor"=refnum, "Calibration Type"=refnum, "Show Line"=refnum, "Phase Lifetime 1"=refnum, "Phase Lifetime 2"=refnum, "Phasor Graph Frequency"=refnum, "Phasor Reference 1 Control"=refnum, "Phasor Reference 2 Control"=refnum, "Calibration Lifetime"=refnum, "Phase Lifetime SDV"=refnum, "Average Lifetime SDV"=refnum, "Phasor Ratio SDV"=refnum, "Modulus Lifetime SDV"=refnum, "Phasor Graph"=refnum} ("Phasor Graph Ctrl Refnums"), "Phasor Graph"=w1, "Phasor Ratio"=w32, "Modulus Lifetime"=w31, "Phasor at cursor (m, phi)"=w30, "Phase Lifetime"=w29, "Phasor at cursor (g, s)"=w28, "Phasor Graph Average Lifetime"=w27, "Phasor Graph Active"=w26, "Save Phasor Graph"=w25, "Phasor Frame Slide"=w24, "Single Step Phasor"=w23, "Calibration Type"=w22, "Show Line"=w21, "Phase Lifetime 1"=w20, "Phase Lifetime 2"=w19, "Phasor Graph Frequency"=w18, "Phasor Reference 1 Control"=w11, "Phasor Reference 2 Control"=w17, "Calibration Lifetime"=w16, "Phase Lifetime SDV"=w15, "Average Lifetime SDV"=w14, "Phasor Ratio SDV"=w13, "Modulus Lifetime SDV"=w12) -> (w38:T5)
  n25 = call "AlliGator Refnums Storage.vi"("Get(F)/Set"=TRUE, "AlliGator Refnum List"=AlliGator_Refnums_List."Phasor Graph Ctrl Refnums", "Data in"=w38) -> ("Error Out"=w3:errorcluster)  [unwired: 7 in, 1 out]
  n26 = control-ref of="This VI"() -> (w5:refnum<vi>)
  n27 = call "AlliGator Store VI Refnum.vi"("error in (no error)"=w3, "VI Refnum"=w5) -> ("error out"=w2:errorcluster, "VI Refnum (dup)"=w4:refnum<vi>)  [unwired: 7 in, 1 out]
  n28 = call "Open VI Front Panel Hidden.vi"("error in"=w2, "VI in"=w4) -> ("error out"=w10:errorcluster, "VI out"=w8:refnum<vi>)  [unwired: 8 in]
  n29 = call "AlliGator subPanel User Event Refnum.vi"() -> ("subPanel Event"=w46:refnum<user-event>)  [unwired: 9 in]
  n30 = register-events(error in=w10, w46) -> (reference out=w45:refnum<event-registration>, error out=w9:errorcluster)  [unwired: 1 in]
  n31 = call "XY Graph TipStrip Event Registration.vi"("error in (no error)"=w9, "XY Graph Refnum"=w1) -> ("error out"=w7:errorcluster, "Event Registration Refnum"=w36:refnum<event-registration>)  [unwired: 7 in, 1 out]
  n32 = call "Close Front Panel.vi"("error in (no error)"=w7, "VI in"=w8) -> ("VI out"=w6:refnum<vi>)  [unwired: 8 in, 1 out]
  n33 = call "AlliGator Queue.vi"() -> ("AlliGator Q"=w48:refnum<queue>)  [unwired: 8 in, 1 out]
  n34 = Bundle("Event Registration Refnum"=w45, "Event Registration Refnum"=w36) -> (w37:T6)  [unwired: 1 in]
  n35 = call "Get Notebook Queue.vi"() -> ("Notebook Queue"=w49:refnum<queue>)  [unwired: 9 in]
  n36 = while {
    tunnel: w49 -> [w61]
    tunnel: w48 -> [w58]
    tunnel: "AlliGator" ("Sender") -> [w56]
    tunnel: w6 -> [w54]
    tunnel: w37 -> [w53]
    tunnel: [w52] -> w44
    tunnel: [w51] -> w43
    stop <- w68 stop-if-true
    n37 = call "Busy Icon & Message Storage.vi"() -> ("Busy Icon Status (F = busy)"=w55:bool)  [unwired: 9 in, 2 out]
    n38 = event shown="[25] Panel Close?" {
      selector: w53 -> [_ _ _ _ _ _ _ _ _ _ _ _ _ _ _ _ _ _ _ _ _ _ w317 w322 _ _]
      dyn-events: [_ _ _ _ _ _ _ _ _ _ _ _ _ _ _ _ _ _ _ _ _ _ w315 w320 _ _] -> w52
      timeout: _ -> [_ _ _ _ _ _ _ _ _ _ _ _ _ _ _ _ _ _ _ _ _ _ _ _ _ _]
      tunnel: [_ _ _ _ _ _ _ w144 w149 w177 _ _ _ w213 w232 w250 _ _ _ _ w306 _ _ _ _ w331] -> w62
      tunnel: [_ _ _ _ _ _ _ _ _ _ _ _ _ _ _ _ _ _ _ _ _ w309 _ _ _ _] -> w68
      tunnel: [_ _ _ _ _ _ _ _ w150 _ _ _ _ _ w233 _ _ _ _ _ _ _ _ _ _ _] -> w59
      tunnel: [w69 w78 w105 w111 w121 w126 w134 _ w151 _ w194 w203 w211 _ w234 w251 w267 w279 w293 w303 _ _ _ _ _ _] -> w57
      tunnel: w55 -> [w72 w79 w110 w112 w125 w127 w133 _ _ _ _ w201 w210 _ w236 w249 w265 w278 w294 w302 _ _ _ _ _ _]
      tunnel: w56 -> [_ _ _ _ _ _ _ _ w148 _ _ _ _ _ _ _ _ _ _ _ _ _ _ _ _ _]
      tunnel: w54 -> [_ _ _ _ _ _ _ _ _ _ _ _ _ _ _ _ _ _ _ _ w308 _ _ _ _ w330]
      tunnel: "Busy" ("ItemTag") -> [w71 _ w109 _ w124 _ _ _ _ _ _ _ _ _ _ _ _ _ _ _ _ _ _ _ _ _]
      event "Calibration Lifetime": Shortcut Menu Selection (User) {
        n39 = event-data() -> ("ItemTag"=w73:string)  [unwired: 1 in]
        n40 = Select(t=w73, s=w72, f=w71) -> (s? t:f=w70:string)
        n41 = case shown="Default" w70 {
          tunnel: [_ w74 w76] -> w69
          frame Default {
          }
          frame "Use as Phasor Reference 1 Lifetime" {
            n42 = Build Array(T8 {"AlliGator Q Event"=enum."Phasor Ratio:Use as Phasor Reference 1 Lifetime", "Data"=variant} ("element")) -> (w74:T8[])
          }
          frame "Use as Phasor Reference 2 Lifetime" {
            n43 = Build Array(T8 {"AlliGator Q Event"=enum."Phasor Ratio:Use as Phasor Reference 2 Lifetime", "Data"=variant} ("element")) -> (w76:T8[])
          }
        }
      }
      event Value Change {
        n44 = event-data() -> ("CtlRef"=w82:refnum<vi>, "OldVal"=w81:T1, "NewVal"=w80:T1)  [unwired: 1 in]
        n45 = case shown="True" w79 {
          tunnel: w82 -> [w84 _]
          tunnel: w81 -> [w83 _]
          tunnel: w80 -> [_ w93]
          tunnel: [_ w89] -> w78
          frame False {
            n46 = property class="Enum (strict)"(reference=w84, "Value"=w83) -> ()  [unwired: 1 in, 2 out]
          }
          frame True {
            n47 = call "AlliGator Refnums Storage.vi"("AlliGator Refnum List"=AlliGator_Refnums_List."AlliGator Menu") -> ("Error Out"=w85:errorcluster, "Data out"=w87:variant)  [unwired: 9 in]
            n48 = Variant To Data(error in=w85, Variant=w87) -> (data=w86:refnum<k9>)  [unwired: 1 in, 1 out]
            n49 = Bundle By Name(cluster=T8 {"AlliGator Q Event"=enum."Calibration:Set Calibration Type", "Data"=variant} ("element"), "Data"=w93) -> (w94:T8)
            n50 = case shown="\"Phasor Map\"" w93 {
              tunnel: [_ TRUE ("Use Calibration Phasor") FALSE ("Use Calibration Phasor") FALSE ("Use Calibration Phasor")] -> w92
              tunnel: [_ FALSE ("Use Calibration Phasor Curve") TRUE ("Use Calibration Phasor Curve") FALSE ("Use Calibration Phasor Curve")] -> w91
              tunnel: [_ FALSE ("Use Calibration Phasor Map") FALSE ("Use Calibration Phasor Map") TRUE ("Use Calibration Phasor Map")] -> w90
              frame "None", Default {
              }
              frame "Single Phasor" {
              }
              frame "Phasor Series" {
              }
              frame "Phasor Map" {
              }
            }
            n51 = Build Array(w94) -> (w89:T8[])
            n52 = call "AlliGator Check Calibration Menu Items.vi"("Use Calibration Phasor Map"=w90, "Use Calibration Phasor Curve"=w91, "Use Calibration Phasor"=w92, "Menu in"=w86) -> ()  [unwired: 7 in, 1 out]
          }
        }
      }
      event Shortcut Menu Selection (User) {
        n53 = event-data() -> ("CtlRef"=w108:refnum<vi>, "ItemTag"=w106:string)  [unwired: 1 in]
        n54 = Select(t=w106, s=w110, f=w109) -> ()  [unwired: 1 out]
        n55 = property class="Clust (strict)"(reference=w108) -> ("Value"=w107:T3)  [unwired: 1 in, 2 out]
        n56 = call "AlliGator Current Phasor (g, s) Custom Menu Actions.vi"("Menu Item Tag"=w106, "Current Phasor"=w107) -> ("AlliGator Actions"=w105:T8[])  [unwired: 9 in]
      }
      event Value Change {
        n57 = event-data() -> ("NewVal"=w113:T3)  [unwired: 1 in]
        n58 = case shown="True" w112 {
          tunnel: w113 -> [_ w116]
          tunnel: [_ w115] -> w111
          frame False {
          }
          frame True {
            n59 = Build Array(w116) -> (w114:T3[])
            n60 = Bundle By Name(cluster=T8 {"AlliGator Q Event"=enum."Phasor Graph:Update Last Phasor Value", "Data"=variant} ("element"), "Data"=w114) -> (w117:T8)
            n61 = Build Array(w117) -> (w115:T8[])
          }
        }
      }
      event Shortcut Menu Selection (User) {
        n62 = event-data() -> ("CtlRef"=w123:refnum<vi>, "ItemTag"=w122:string)  [unwired: 1 in]
        n63 = Select(t=w122, s=w125, f=w124) -> ()  [unwired: 1 out]
        n64 = property class="Clust (strict)"(reference=w123) -> ("Value"=w120:T2)  [unwired: 1 in, 2 out]
        n65 = call "Phasor Convert (m, phi) to (g,s).vi"("Phasor (m, phi)"=w120) -> ("Phasor (g, s)"=w119:T3)  [unwired: 8 in]
        n66 = call "AlliGator Current Phasor (g, s) Custom Menu Actions.vi"("Menu Item Tag"=w122, "Current Phasor"=w119) -> ("AlliGator Actions"=w121:T8[])  [unwired: 9 in]
      }
      event Value Change {
        n67 = event-data() -> ("NewVal"=w128:T2)  [unwired: 1 in]
        n68 = case shown="True" w127 {
          tunnel: w128 -> [_ w130]
          tunnel: [_ w129] -> w126
          frame False {
          }
          frame True {
            n69 = Bundle By Name(cluster=T8 {"AlliGator Q Event"=enum."Phasor Graph:Update Phasor (m, phi)", "Data"=variant} ("element"), "Data"=w130) -> (w131:T8)
            n70 = Build Array(w131) -> (w129:T8[])
          }
        }
      }
      event "Phasor Frame Slide": Value Change {
        n71 = event-data() -> ("CtlRef"=w137:refnum<vi>, "OldVal"=w136:i32, "NewVal"=w135:i32)  [unwired: 1 in]
        n72 = case shown="True" w133 {
          tunnel: w135 -> [_ w141]
          tunnel: w137 -> [w139 _]
          tunnel: w136 -> [w138 _]
          tunnel: [_ w140] -> w134
          frame False {
            n73 = property class="Slide (strict)"(reference=w139, "Value"=w138) -> ()  [unwired: 1 in, 2 out]
          }
          frame True {
            n74 = Bundle By Name(cluster=T8 {"AlliGator Q Event"=enum."Phasor Graph:Show Single Phasor", "Data"=variant} ("element"), "Data"=w141) -> (w142:T8)
            n75 = Build Array(w142) -> (w140:T8[])
          }
        }
      }
      event "Phasor Graph Active": Value Change {
        n76 = event-data() -> ("NewVal"=w145:bool)  [unwired: 1 in]
        n77 = call "AlliGator Settings Storage.vi"("Get(F)/Set"=TRUE, "AlliGator Settings List"=AlliGator_Settings_List."Phasor Graph:Phasor Graph Active", "Variant Data in"=w145) -> ("Error Out"=w144:errorcluster)  [unwired: 7 in, 1 out]
      }
      event "Phasor Graph Frequency", "Save Phasor Graph Image", "Calibration Lifetime": Value Change {
        n78 = event-data() -> ("CtlRef"=w153:refnum<vi>)  [unwired: 1 in]
        n79 = property class="Ctl"(reference=w153) -> (reference out=w156:refnum<vi>, error out=w155:errorcluster, "Label.Text"=w152:string, "Value"=w154:variant)  [unwired: 1 in]
        n80 = case shown="\"Phasor Graph Frequency\"" w152 {
          tunnel: w155 -> [w159 w160 w172]
          tunnel: [w159 w161 w174] -> w157
          tunnel: [_ _ w176] -> w151
          tunnel: w148 -> [_ _ w175]
          tunnel: w154 -> [_ _ w173]
          frame "", Default {
            # "only updates the corresponding Settings window control"
          }
          frame "Calibration Lifetime" {
            n81 = disable-structure shown="Disabled" {
              disable-tunnel: [w164 _] -> w161
              disable-tunnel: w160 -> [w163 _]
              frame Disabled {
                n82 = call "Alligator Variables Storage.vi"("AlliGator Variable"=AlliGator_Variables_List."Phasor Plot:Computed" ("Alligator Variable"), "Error In"=w163) -> ("Error Out"=w162:errorcluster, "Data out"=w166:variant)  [unwired: 7 in, 1 out]
                n83 = call-poly "Variant to Data.vi"("Variant"=w166) -> ("Value"=w165:bool)  [unwired: 8 in]
                n84 = case shown="True" w165 {
                  tunnel: w162 -> [w168 w171]
                  tunnel: [w168 w169] -> w164
                  frame False {
                  }
                  frame True {
                    n85 = call "AlliGator Set Phasor Plot Update LED.vi"("error in (no error)"=w171, "Off/On"=TRUE) -> ("error out"=w169:errorcluster)  [unwired: 9 in]
                  }
                }
              }
              frame Enabled {
              }
            }
          }
          frame "Phasor Graph Frequency" {
            n86 = call "AlliGator Phasor Graph Update Phasor Frequency.vi"("error in (no error)"=w172, "Value"=w173, "Sender"=w175) -> ("error out"=w174:errorcluster, "AlliGator Q Elements"=w176:T8[])  [unwired: 7 in]
          }
        }
        n87 = call "AlliGator Update Settings & Control.vi"("Error In"=w157, "Value"=w154, "Sender"=w148, "CtlRef"=w156) -> ("Error Out"=w158:errorcluster)  [unwired: 7 in]
        n88 = call "AlliGator Get Control Notebook String.vi"("error in (no error)"=w158, "Value"=w154, "Control Label"=w152) -> ("error out"=w149:errorcluster, "Notebook String"=w150:string)  [unwired: 7 in]
      }
      event "Phasor Graph Frequency": Shortcut Menu Selection (User) {
        n89 = event-data() -> ("CtlRef"=w179:refnum<vi>, "ItemTag"=w178:string)  [unwired: 1 in]
        n90 = case shown="\"\", Default" w178 {
          tunnel: w179 -> [_ w181 w184 w187 w191]
          tunnel: [_ w180 w182 w185 w188] -> w177
          frame "", Default {
          }
          frame "f = 1/T" {
            n91 = call "AlliGator Set Phasor Harmonic.vi"("Phasor Frequency Refnum"=w181) -> ("Error Out"=w180:errorcluster)  [unwired: 10 in]
          }
          frame "f = 1/D" {
            n92 = call "AlliGator Set Phasor Harmonic.vi"("Use n/D"=TRUE, "Phasor Frequency Refnum"=w184) -> ("Error Out"=w182:errorcluster)  [unwired: 9 in]
          }
          frame "f = n/T (n > 1)" {
            n93 = call "AlliGator Set Phasor Harmonic.vi"("Harmonic (1)"=0, "Phasor Frequency Refnum"=w187) -> ("Error Out"=w185:errorcluster)  [unwired: 9 in]
          }
          frame "f = n/D (n > 1)" {
            n94 = call "AlliGator Set Phasor Harmonic.vi"("Use n/D"=TRUE, "Harmonic (1)"=0, "Phasor Frequency Refnum"=w191) -> ("Error Out"=w188:errorcluster)  [unwired: 8 in]
          }
        }
      }
      event "Phasor Graph": event #0x4e {
        n95 = event-data() -> ("ItemTag"=w195:string, "CtlRef"=w196:refnum<vi>, "Coords"=w193:T12, "ItemPath"=w192:string)  [unwired: 1 in]
        n96 = case shown="\"CURS_FREE\", \"CURS_MULTI\", \"CURS_SINGLE\"" w195 {
          tunnel: w196 -> [_ w197]
          tunnel: [_ w199] -> w194
          tunnel: w193 -> [_ _]
          tunnel: w192 -> [_ _]
          frame "", Default {
          }
          frame "CURS_FREE", "CURS_MULTI", "CURS_SINGLE" {
            n97 = Bundle By Name(cluster=T8 {"AlliGator Q Event"=enum."Generic Graph:Set Last Cursor Style", "Data"=variant} ("AlliGator Actions"), "Data"=w197) -> (w198:T8)
            n98 = Build Array(w198) -> (w199:T8[])
          }
        }
      }
      event "Phasor Graph": Cursor Move {
        n99 = event-data() -> ("Time"=w202:u32)  [unwired: 1 in]
        n100 = case shown="True" w201 {
          tunnel: [_ w207] -> w203
          tunnel: w202 -> [_ w205]
          frame False {
          }
          frame True {
            w206 = T8 {"AlliGator Q Event"=enum."Phasor Graph:Cursor Move", "Data"=variant} ("Time-Gated Phasor Q Element")
            n101 = call "AlliGator Filter Event.vi"("Time"=w205, "AlliGatorr Q Element"=w206) -> ("Filter Event?"=w204:bool)  [unwired: 8 in, 1 out]
            n102 = case shown="False" w204 {
              tunnel: w206 -> [w209 _]
              tunnel: [w208 _] -> w207
              frame False {
                n103 = Build Array(w209) -> (w208:T8[])
              }
              frame True {
              }
            }
          }
        }
      }
      event "Phasor Graph": Scale Range Change; "Phasor Graph": Autoscale Range Change; "Phasor Graph": Cursor Release {
        n104 = event-data() -> ()  [unwired: 1 in, 4 out]
        n105 = case shown="True" w210 {
          tunnel: [_ T8[] [{"AlliGator Q Event"=enum."Phasor Graph:Draw Cursor Connecting Line", "Data"=variant}] ("element")] -> w211
          frame False {
          }
          frame True {
          }
        }
      }
      event "Phasor Graph": Shortcut Menu Activation? {
        n106 = event-data() -> ("CtlRef"=w215:refnum<vi>, "MenuRef"=w214:refnum<k9>)  [unwired: 1 in]
        n107 = call "XY Graph Check-Uncheck Menu Items.vi"("Menu in"=w214, "XY Graph Refnum"=w215) -> ("Error Out (dup)"=w224:errorcluster, "Menu out"=w219:refnum<k9>, "XY Graph Refnum dup"=w217:T14)  [unwired: 6 in, 1 out]
        n108 = call "XY Graph Get Label.vi"("XYGraph"=w217) -> ("Graph Label"=w216:string)  [unwired: 8 in]
        n109 = case shown="\"\", Default" w216 {
          tunnel: w224 -> [w225 w231]
          tunnel: [w225 w230] -> w220
          tunnel: w219 -> [w226 w229]
          tunnel: [w226 w228] -> w218
          frame "", Default {
          }
          frame "Decay Graph" {
            n110 = call "AlliGator Decay Graph Get-Set Process Plot Target.vi"("Get (F)/Set"=FALSE, "Error In"=w231, "Menu"=w229) -> ("Error Out (dup)"=w230:errorcluster, "Menu"=w228:refnum<k9>)  [unwired: 6 in, 1 out]
          }
        }
        n111 = call "AlliGator Add Python Functions to Object Menu.vi"("error in (no error)"=w220, "Menu in"=w218, "Object Refnum"=w217) -> ("error out"=w223:errorcluster, "Menu out"=w222:refnum<k9>, "Object Refnum dup"=w221:refnum<vi>)  [unwired: 6 in]
        n112 = call "AlliGator Grayed out Menu Items.vi"("error in (no error)"=w223, "Menu in"=w222, "Object Refnum"=w221) -> ("error out"=w213:errorcluster)  [unwired: 7 in, 1 out]
        n113 = event-data() -> ()  [unwired: 2 in, 1 out]
      }
      event "Phasor Graph": Shortcut Menu Selection (User) {
        n114 = event-data() -> ("CtlRef"=w238:refnum<vi>, "Coords"=w241:T12, "ItemTag"=w239:string, "ItemPath"=w240:string)  [unwired: 1 in]
        n115 = call "AlliGator Keyboard ID.vi"() -> ("keys pressed"=w245:T15)  [unwired: 9 in, 2 out]
        n116 = Bundle By Name(cluster=T11 {"Item Tag"="", "XY Graph Refnum"=refnum, "Coords"={"Horizontal"=0, "Vertical"=0}, "Item Path"=""} ("XY Graph Event"), "XY Graph Refnum"=w238, "Coords"=w241, "Item Tag"=w239, "Item Path"=w240) -> (w237:T11)
        n117 = Index Array(array=w245) -> (element=w242:T13)  [unwired: 1 in]
        n118 = Equal?(x=w242, y=T13."H" ("element")) -> (x = y?=w235:bool)
        n119 = call "AlliGator Phasor Graph Context Menu Handler.vi"("Help?"=w235, "Animated Busy Icon"=w236, "XY Graph Event"=w237) -> ("Error Out"=w232:errorcluster, "Message"=w233:string, "AlliGator Actions"=w234:T8[])  [unwired: 6 in]
      }
      event "Show Line": Value Change {
        n120 = event-data() -> ("CtlRef"=w248:refnum<vi>, "NewVal"=w247:bool, "OldVal"=w246:bool)  [unwired: 1 in]
        n121 = case shown="True" w249 {
          tunnel: w248 -> [w254 _]
          tunnel: w247 -> [_ w257]
          tunnel: w246 -> [w253 _]
          tunnel: [w252 w256] -> w250
          tunnel: [_ w258] -> w251
          frame False {
            n122 = property class="Bool (strict)"(reference=w254, "Value"=w253) -> (error out=w252:errorcluster)  [unwired: 1 in, 1 out]
          }
          frame True {
            n123 = call "Alligator Variables Storage.vi"("AlliGator Variable"=AlliGator_Variables_List."Phasor Graph:Show Line", "Data in"=w257) -> ("Error Out"=w256:errorcluster)  [unwired: 7 in, 2 out]
            n124 = Build Array(T8 {"AlliGator Q Event"=enum."Phasor Graph:Draw Cursor Connecting Line", "Data"=variant} ("Time-Gated Phasor Q Element"), T8 {"AlliGator Q Event"=enum."Phasor Graph:Find UC Intersection", "Data"=variant} ("Time-Gated Phasor Q Element")) -> (w260:T8[])
            n125 = Select(t=w260, s=w257, f=T8[] [{"AlliGator Q Event"=enum."Phasor Graph:Clear Cursor Connecting Line", "Data"=variant}] ("element")) -> (s? t:f=w258:T8[])
          }
        }
      }
      event "Single Step Phasor": Value Change {
        n126 = event-data() -> ("CtlRef"=w266:refnum<vi>, "NewVal"=w264:bool, "OldVal"=w263:bool)  [unwired: 1 in]
        n127 = case shown="True" w265 {
          tunnel: w264 -> [_ w271]
          tunnel: w266 -> [w269 _]
          tunnel: w263 -> [w268 _]
          tunnel: [_ w272] -> w267
          frame False {
            n128 = property class="Bool (strict)"(reference=w269, "Value"=w268) -> ()  [unwired: 1 in, 2 out]
          }
          frame True {
            n129 = property on="Phasor Frame Slide" class="Slide (strict)"("Visible"=w271) -> ("Value"=w270:i32)  [unwired: 2 in, 2 out]
            n130 = Select(t=w270, s=w271, f=0) -> (s? t:f=w274:i32)
            n131 = Decrement(x=w274) -> (x-1=w273:i32)
            n132 = Bundle By Name(cluster=T8 {"AlliGator Q Event"=enum."Phasor Graph:Show Single Phasor", "Data"=variant} ("element"), "Data"=w273) -> (w276:T8)
            n133 = Build Array(w276) -> (w272:T8[])
          }
        }
      }
      event "Phasor Reference 1 Control": Value Change {
        n134 = event-data() -> ("CtlRef"=w282:refnum<vi>, "OldVal"=w281:dbl, "NewVal"=w280:dbl)  [unwired: 1 in]
        n135 = case shown="True" w278 {
          tunnel: w280 -> [_ w287]
          tunnel: w282 -> [w284 _]
          tunnel: w281 -> [w283 _]
          tunnel: [_ w285] -> w279
          frame False {
            n136 = property class="Scroll (strict)"(reference=w284, "Value"=w283) -> ()  [unwired: 1 in, 2 out]
          }
          frame True {
            n137 = Bundle By Name(cluster=T8 {"AlliGator Q Event"=enum."Phasor Ratio:Update Phasor Reference 1", "Data"=variant} ("Time-Gated Phasor Q Element"), "Data"=w287) -> (w288:T8)
            n138 = Build Array(w288, T8 {"AlliGator Q Event"=enum."Phasor Graph:Draw Cursor Connecting Line", "Data"=variant} ("Time-Gated Phasor Q Element")) -> (w285:T8[])
          }
        }
      }
      event "Phasor Reference 2 Control": Value Change {
        n139 = event-data() -> ("CtlRef"=w292:refnum<vi>, "OldVal"=w291:dbl, "NewVal"=w290:dbl)  [unwired: 1 in]
        n140 = case shown="True" w294 {
          tunnel: w290 -> [_ w299]
          tunnel: w292 -> [w296 _]
          tunnel: w291 -> [w295 _]
          tunnel: [_ w297] -> w293
          frame False {
            n141 = property class="Scroll (strict)"(reference=w296, "Value"=w295) -> ()  [unwired: 1 in, 2 out]
          }
          frame True {
            n142 = Bundle By Name(cluster=T8 {"AlliGator Q Event"=enum."Phasor Ratio:Update Phasor Reference 2", "Data"=variant} ("Time-Gated Phasor Q Element"), "Data"=w299) -> (w300:T8)
            n143 = Build Array(w300, T8 {"AlliGator Q Event"=enum."Phasor Graph:Draw Cursor Connecting Line", "Data"=variant} ("Time-Gated Phasor Q Element")) -> (w297:T8[])
          }
        }
      }
      event "Refresh SEPL": Value Change {
        n144 = event-data() -> ()  [unwired: 1 in, 1 out]
        n145 = case shown="True" w302 {
          tunnel: [_ w304] -> w303
          frame False {
          }
          frame True {
            n146 = Build Array(T8 {"AlliGator Q Event"=enum."Phasor Graph:Update SEPL Plot", "Data"=variant} ("element")) -> (w304:T8[])
          }
        }
      }
      event "Pin Button": Value Change {
        n147 = event-data() -> ("NewVal"=w307:bool)  [unwired: 1 in]
        n148 = call "AlliGator Dock-Undock Subpanel Event.vi"("Dock?"=w307, "VI in"=w308) -> ("Error Out"=w306:errorcluster)  [unwired: 9 in]
      }
      event User Event {
        n149 = event-data() -> ("subpanel"=w311:string, "event"=w310:string)  [unwired: 1 in]
        n150 = case shown="\"AlliGator\"" w311 {
          tunnel: w310 -> [_ w313]
          tunnel: [_ w312] -> w309
          frame "False", Default {
          }
          frame "AlliGator" {
            n151 = case shown="\"False\", Default" w313 {
              tunnel: [_ TRUE] -> w312
              frame "False", Default {
              }
              frame "quit" {
              }
            }
          }
        }
      }
      event Mouse Enter {
        n152 = event-data() -> ("CtlRef"=w316:refnum<vi>)  [unwired: 1 in]
        n153 = Unbundle By Name(w317) -> ("Event Registration Refnum"=w319:refnum<event-registration>)
        n154 = call "XY Graph Tipstrip Mouse Enter.vi"("Event Registration Refnum"=w319, "XY Graph Refnum"=w316) -> ("Event Registration Refnum"=w318:refnum<event-registration>)  [unwired: 8 in, 1 out]
        n155 = Bundle By Name(cluster=w317, "Event Registration Refnum"=w318) -> (w315:T6)
      }
      event Mouse Leave {
        n156 = event-data() -> ("CtlRef"=w321:refnum<vi>)  [unwired: 1 in]
        n157 = Unbundle By Name(w322) -> ("Event Registration Refnum"=w323:refnum<event-registration>)
        n158 = call "XY Graph Tipstrip Mouse Leave.vi"("Event Registration Refnum"=w323, "XY Graph Refnum"=w321) -> ("Event Registration Refnum"=w324:refnum<event-registration>)  [unwired: 8 in, 1 out]
        n159 = Bundle By Name(cluster=w322, "Event Registration Refnum"=w324) -> (w320:T6)
      }
      event Mouse Move {
        n160 = event-data() -> ("CtlRef"=w327:refnum<vi>, "Coords"=w326:T12)  [unwired: 1 in]
        n161 = control-ref of="Phasor Graph TipStrip"() -> (w325:refnum<vi>)
        n162 = call "XY Graph Set Plot TipStrip.vi"("TipStrip Refnum"=w325, "Max Length (200)"=300, "Coords"=w326, "XY Graph Refnum"=w327) -> ()  [unwired: 5 in, 3 out]
      }
      event Panel Close? {
        w329 = TRUE ("Pin Button")
        n163 = event-data() -> ()  [unwired: 1 in, 1 out]
        n164 = property on="Pin Button" class="Bool (strict)"("Value"=w329) -> (error out=w332:errorcluster)  [unwired: 2 in, 1 out]
        n165 = call "AlliGator Dock-Undock Subpanel Event.vi"("Error In"=w332, "Dock?"=w329, "VI in"=w330) -> ("Error Out"=w331:errorcluster)  [unwired: 8 in]
        n166 = event-data("Discard?"=w329) -> ()  [unwired: 1 in, 1 out]
      }
    }
    n167 = call "AlliGator Settings Storage.vi"("AlliGator Settings List"=AlliGator_Settings_List."Miscellaneous:Verbose Error Mode") -> ("Variant Data out"=w67:variant)  [unwired: 9 in, 1 out]
    n168 = call-poly "Variant to Data.vi"("Variant"=w67) -> ("Value"=w60:bool)  [unwired: 8 in]
    n169 = call "Send Message to Notebook.vi"("Error In"=w62, "Text"=w59, "Notebook Queue"=w61) -> ("Error Out"=w64:errorcluster, "Notebook Queue"=w63:refnum<queue>)  [unwired: 5 in]
    n170 = call "Light Theme Message Style.vi"() -> ()  [unwired: 1 out]
    n171 = call "AlliGator Queue Non Empty Events.vi"("Actions"=w57, "AlliGator Q"=w58) -> ()  [unwired: 9 in, 1 out]
    n172 = call "Send Error to Notebook.vi"("error in (no error)"=w64, "Verbose Error Messages (T)"=w60, "State Machine Case Error Source"="Phasor Graph", "Notebook Q"=w63) -> ("Error Out"=w51:errorcluster)  [unwired: 7 in]
  }
  n173 = call "Tiny Clear Error.vi"("Error In"=w43) -> ("no Error Out"=w42:errorcluster)  [unwired: 8 in]
  n174 = Unregister For Events(event registration refnum=w44) -> (error out=w34:errorcluster)  [unwired: 1 in]
  n175 = invoke class="VI" method="FP.Close"(reference=w6, error in=w42) -> (error out=w35:errorcluster)  [unwired: 1 in, 2 out]
  n176 = Merge Errors(w35, w34) -> (w33:errorcluster)
  n177 = call "Tiny Clear Error.vi"("Error In"=w33) -> ()  [unwired: 8 in, 1 out]
